vi "Analysis Produces Correct number of Functions.vi"(11 "Test Case In":refnum<class "Python Code Analysis.lvclass">) -> (0 "error out":errorcluster, 3 "Test Case Out":refnum<class "Python Code Analysis.lvclass">)   [LabVIEW 2026, in "Python Code Analysis.lvclass"]
doc: "This tests that the analysis of the dummy python module produces the correct amount of functions."
uses:
  Python Code Analysis.lvclass
  C:/Program Files/National Instruments/LabVIEW 2026/vi.lib/Astemes/LUnit/Test Case.lvclass
  <vilib>/Astemes/LUnit/Test Case.lvclass/Test Case.ctl
  <vilib>/Astemes/LUnit/Core/LUnit Test Case/Private/Append Fail Result.vi
  <vilib>/Astemes/LUnit/Core/LUnit Test Case/Private/Append Pass Result.vi
  <vilib>/Astemes/LUnit/Core/LUnit Test Case/Private/Run In UI.vi
  <vilib>/Utility/error.llb/Clear Errors.vi
  Python Code Analysis.lvclass/Python Code Analysis.ctl
  <vilib>/Astemes/LUnit/Test Case.lvclass
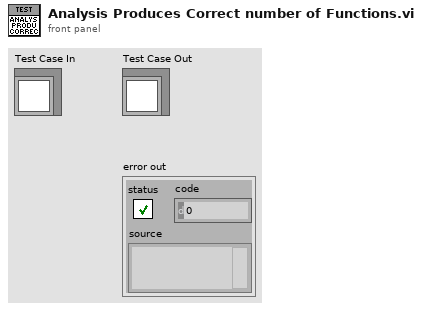
[diagram p1: front panel]
types:
  T1 = typedef "Analysis Output--cluster.ctl" = cluster{"type_definitions":T2[], "functions":T4[]}
  T2 = typedef "Type Definition--cluster.ctl" = cluster{"name":string, "fields":T3[]}
  T3 = typedef "Parameter--cluster.ctl" = cluster{"name":string, "data_type":string, "container":string, "dimensions":i32, "type_definition":string}
  T4 = typedef "Function--cluster.ctl" = cluster{"name":string, "docstring":string, "input_parameters":T3[], "output_parameters":T3[]}
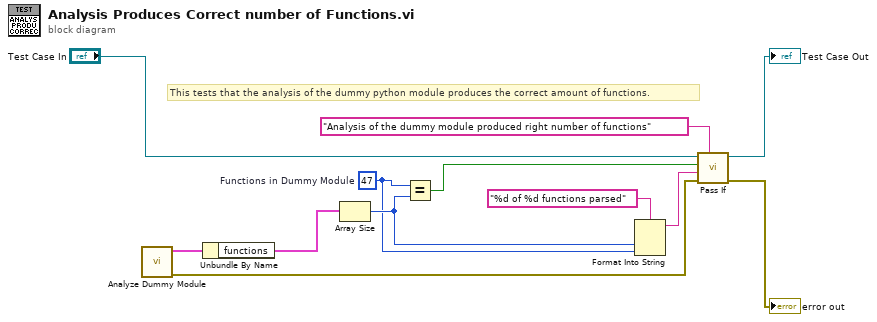
[diagram p0: block diagram]
diagram:
  w5 = 47  # Functions in Dummy Module
  # "This tests that the analysis of the dummy python module produces the correct amount of functions."
  n1 = call "Analyze Dummy Module.vi"() -> ("error out"=w12:errorcluster, "Analysis Output"=w9:T1)  [unwired: 10 in]
  n2 = Unbundle By Name(w9) -> ("functions"=w10:T4[])
  n3 = Array Size(array=w10) -> (size(s)=w6:i32)
  n4 = Equal?(x=w5, y=w6) -> (x = y?=w8:bool)
  n5 = Format Into String(format string="%d of %d functions parsed", w6, w5) -> (resulting string=w4:string)  [unwired: 2 in, 1 out]
  n6 = call <vilib>:"Pass If.vi"("Description"="Analysis of the dummy module produced right number of functions", "error in (no error)"=w12, "Message"=w4, "Pass?"=w8, "LUnit Test Case In"="Test Case In") -> ("error out"=→"error out":errorcluster, "LUnit Test Case Out"=→"Test Case Out":refnum<class "Python Code Analysis.lvclass">)  [unwired: 5 in]
